vi "S_ASD Each Burst SAVE Modified_MS VI.vi"(5 "BL and Raw":T4, 7 "BCC":T1, 8 "error in":errorcluster, 9 "Under D array":T5, 10 "Burst Array":T2, 11 "Filename":path) -> (0 "error out":errorcluster, 2 "R Burst#":i32, 3 "B Table":string[][](table))   [LabVIEW 2018]
uses:
  <vilib>/Analysis/baseanly.llb/Multimode.vi
  <vilib>/Utility/file.llb/Write Delimited Spreadsheet (DBL).vi
  <vilib>/Analysis/NI_AALBase.lvlib
panel:
  out "Estimated BL":dbl[](array[numeric])
  out "B#":i32
  out "Signal# Sum":i32
  out "Burst#Sum Pre":i32
  out "B STD (pA)":dbl
  out "B BL (pA)":dbl
  out "R STD (pA)":dbl
  out "R BL (pA)":dbl
  out "BR TL Point":i32
  out "F ex Info":T3
  out "Burst time length":dbl[](array[numeric])
  in  "Flit Rank":i32=15
  out "LL BR number (n)":i32
  out "BR I-t profie":cluster{dbl[], dbl[]}[](graph)
  out "BR time length (ms)":dbl
  out "BR End time (s)":dbl
  out "BR Start time (s)":dbl
  out "BR number (n)":dbl
  out "REnd time":dbl[](array[numeric])
  out "RStart time":dbl[](array[numeric])
  out "Region Raw data":dbl[](array[numeric])
  out "BR Histogram Graph":T6(graph) caption="ヒストグラムグラフ"
  out "サイズ":i32
  out "BR END IDX":i32
  out "BR Start IDX":i32
  out "A New folder":string
  out "LL BR time length (ms)":dbl
  out "Rigon#":i32
  out "BSX Pass":path
  out "B Region":dbl[](array[numeric])
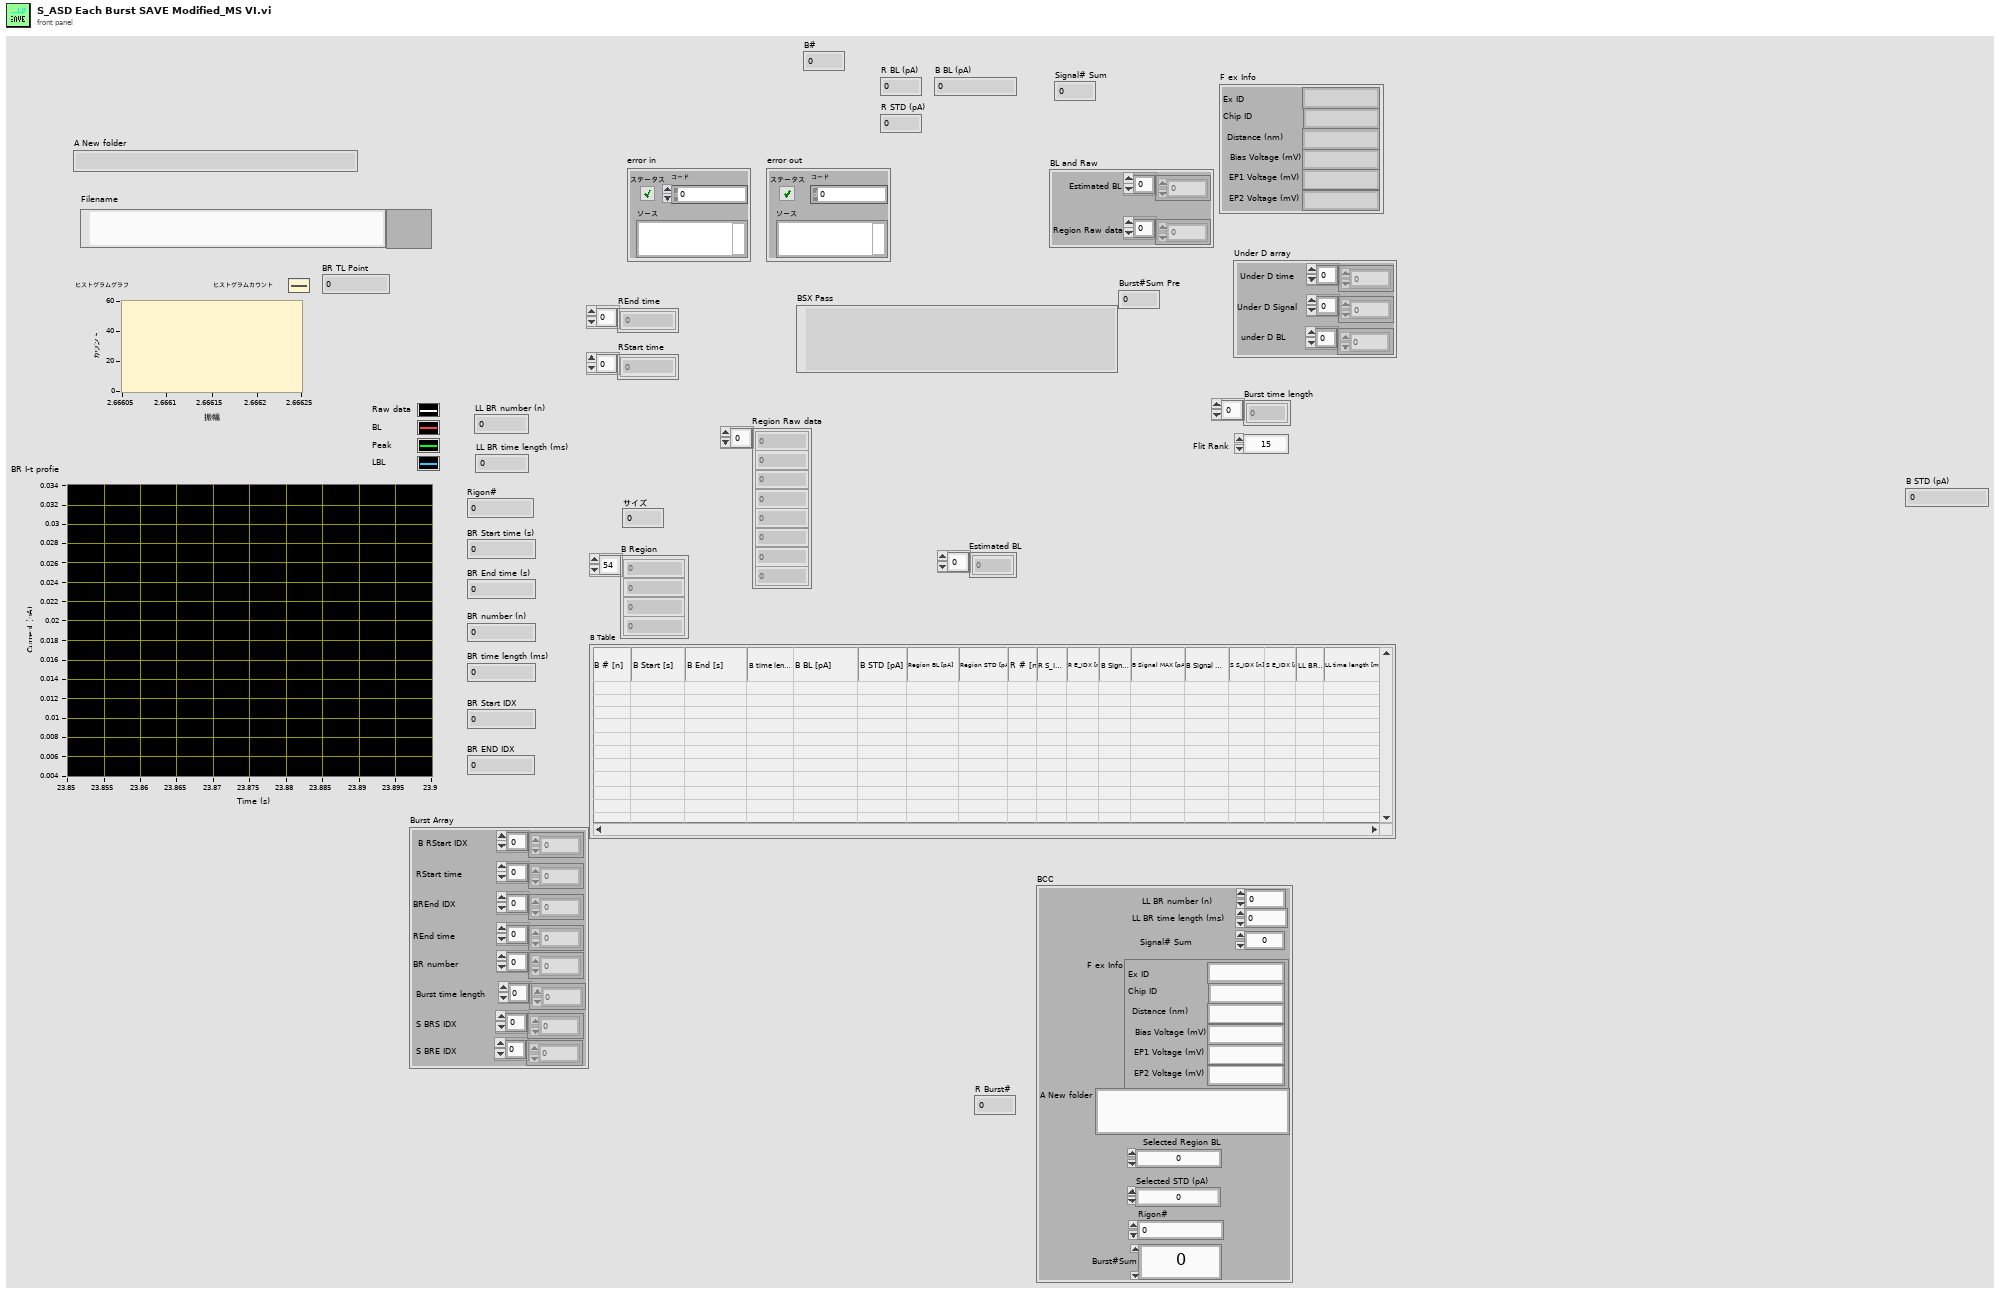
[diagram p1: front panel]
types:
  T1 = cluster{"LL BR number (n)":i32, "LL BR time length (ms)":dbl, "Signal# Sum":i32, "F ex Info":cluster{"Ex ID":string, "Chip ID":string, "Distance (nm)":string, "Bias Voltage (mV)":string, "EP1 Voltage (mV)":string, "EP2 Voltage (mV)":string}, "A New folder":string, "Selected STD (pA)":dbl, "Selected Region BL":dbl, "Rigon#":i32, "Burst#Sum":i32}
  T2 = cluster{"B RStart IDX":i32[], "RStart time":dbl[], "BREnd IDX":i32[], "REnd time":dbl[], "BR number":dbl[], "Burst time length":dbl[], "S BRS IDX":i32[], "S BRE IDX":i32[]}
  T3 = cluster{"Ex ID":string, "Chip ID":string, "Distance (nm)":string, "Bias Voltage (mV)":string, "EP1 Voltage (mV)":string, "EP2 Voltage (mV)":string}
  T4 = cluster{"Estimated BL":dbl[], "Region Raw data":dbl[]}
  T5 = cluster{"Under D time":dbl[], "Under D Signal":dbl[], "under D BL":dbl[]}
  T6 = cluster{"X Values":dbl[], "Histogram: h(x)":i32[]}
  T7 = cluster{"B Under D time":dbl[], "B Under D Signal ":dbl[], "B Under D IDX":i32[], "B Under D BL":dbl[]}
  T8 = cluster{"Size":string, "SH1":string, "SH2":string}
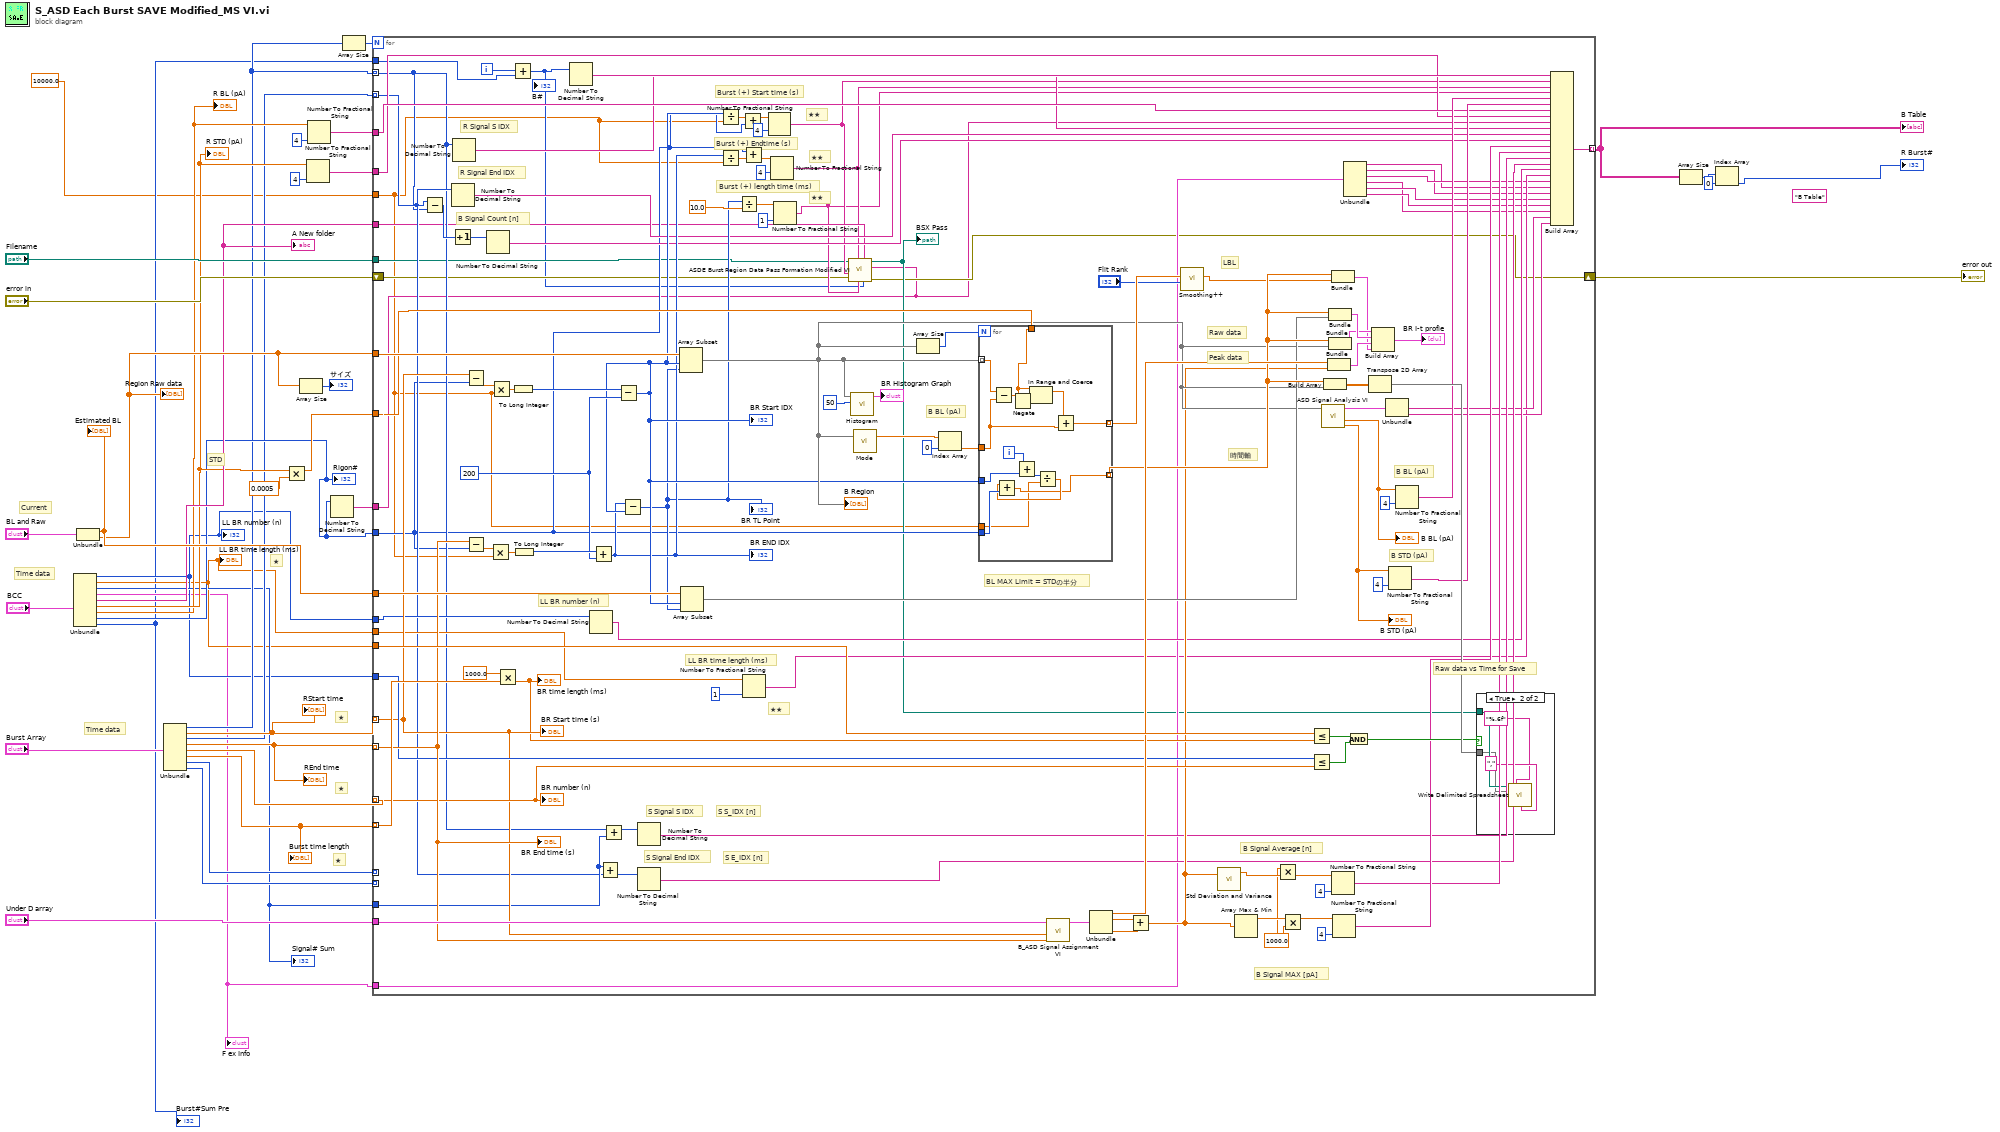
[diagram p0: block diagram]
diagram:
  (unwired) "B Table" ("Group name")
  # "★"
  # "★"
  # "★"
  # "★"
  # "Time data"
  # "Time data"
  # "Current"
  # "STD"
  n1 = Unbundle("BCC") -> ("LL BR number (n)"=w9:i32, "LL BR time length (ms)"=w8:dbl, "Signal# Sum"=w10:i32, "F ex Info"=w7:T3, "A New folder"=w23:string, "Selected STD (pA)"=w20:dbl, "Selected Region BL"=w19:dbl, "Rigon#"=w18:i32, "Burst#Sum"=w6:i32)
  "Rigon#" <- w18
  "LL BR time length (ms)" <- w8
  "A New folder" <- w23
  "LL BR number (n)" <- w9
  "F ex Info" <- w7
  "R BL (pA)" <- w19
  "R STD (pA)" <- w20
  "Burst#Sum Pre" <- w6
  "Signal# Sum" <- w10
  n2 = Unbundle("BL and Raw") -> ("Estimated BL"=w27:dbl[], "Region Raw data"=w26:dbl[])
  "Region Raw data" <- w26
  "Estimated BL" <- w27
  n3 = Unbundle("Burst Array") -> ("B RStart IDX"=w16:i32[], "RStart time"=w33:dbl[], "BREnd IDX"=w17:i32[], "REnd time"=w35:dbl[], "BR number"=w32:dbl[], "Burst time length"=w34:dbl[], "S BRS IDX"=w12:i32[], "S BRE IDX"=w11:i32[])
  "RStart time" <- w33
  "REnd time" <- w35
  "Burst time length" <- w34
  n4 = Multiply(x=w20, y=0.0005) -> (x*y=w30:dbl)
  n5 = Array Size(array=w26) -> (size(s)=→"サイズ":i32)
  n6 = Number To Fractional String(number=w20, precision (6)=i16 4 ("精度（6）")) -> (F-format string=w21:string)  [unwired: 2 in]
  n7 = Number To Fractional String(number=w19, precision (6)=i16 4 ("精度（6）")) -> (F-format string=w22:string)  [unwired: 2 in]
  n8 = Number To Decimal String(number=w18) -> (decimal integer string=w38:string)  [unwired: 1 in]
  n9 = Array Size(array=w16) -> (size(s)=w40:i32)
  n10 = for {
    N: w40 -> [_]
    tunnel: "Filename" -> [w43]
    tunnel: w26 -> [w158]
    tunnel: w38 -> [w47]
    tunnel: w18 -> [w54]
    tunnel: w8 -> [w155]
    shift-right: [w50] -> w2
    shift-left: "error in" -> [w44]
    tunnel: w23 -> [w49]
    tunnel: w33 -> [w113] mode=indexing
    tunnel: w35 -> [w131] mode=indexing
    tunnel: w34 -> [w151] mode=indexing
    tunnel: w32 -> [w129] mode=indexing
    tunnel: w27 -> [w143]
    tunnel: "Under D array" -> [w137]
    tunnel: w9 -> [w130]
    tunnel: w30 -> [w122]
    tunnel: w22 -> [w95]
    tunnel: w21 -> [w94]
    tunnel: w17 -> [w58] mode=indexing
    tunnel: w16 -> [w57] mode=indexing
    tunnel: w12 -> [_] mode=indexing
    tunnel: w11 -> [_] mode=indexing
    tunnel: w6 -> [w78]
    tunnel: w10 -> [w75]
    tunnel: w9 -> [w72]
    tunnel: w8 -> [w70]
    tunnel: w7 -> [w69]
    tunnel: [w60] -> w3 mode=indexing
    tunnel: 10000.0 ("y") -> [w41]
    i -> [w79]
    w82 = 1000.0 ("y")
    w139 = 200 ("S datapoint")
    # "★★"
    # "★★"
    # "★★"
    # "★★"
    # "LL BR time length (ms)"
    # "LL BR number (n)"
    # "S E_IDX [n]"
    # "S S_IDX [n]"
    # "S Signal End IDX"
    # "S Signal S IDX"
    # "B Signal MAX [pA]"
    # "B Signal Average [n]"
    # "B Signal Count [n]"
    # "R Signal End IDX"
    # "R Signal S IDX"
    # "B STD (pA)"
    # "B BL (pA)"
    # "B BL (pA)"
    # "Burst (+) length time (ms)"
    # "Burst (+) Endtime (s)"
    # "Burst (+) Start time (s)"
    # "BL MAX Limit = STDの半分"
    # "Peak data"
    # "Raw data vs Time for Save"
    # "Raw data"
    # "LBL"
    # "時間軸"
    n11 = Subtract(x=w58, y=w57) -> (x-y=w91:i32)
    n12 = Number To Decimal String(number=w58) -> (decimal integer string=w92:string)  [unwired: 1 in]
    n13 = Increment(x=w91) -> (x+1=w90:i32)
    n14 = Number To Decimal String(number=w57) -> (decimal integer string=w93:string)  [unwired: 1 in]
    n15 = Subtract(x=w113, y=w54) -> (x-y=w147:dbl)
    n16 = Subtract(x=w131, y=w54) -> (x-y=w146:dbl)
    n17 = Number To Decimal String(number=w90) -> (decimal integer string=w89:string)  [unwired: 1 in]
    n18 = Multiply(x=w146, y=w41) -> (x*y=w149:dbl)
    n19 = Multiply(x=w147, y=w41) -> (x*y=w150:dbl)
    n20 = Multiply(x=1000.0, y=w151) -> (x*y=w105:dbl)
    "BR time length (ms)" <- w105
    n21 = Add(x=w79, y=w78) -> (x+y=w42:i32)
    "B#" <- w42
    n22 = To Long Integer(number=w150) -> (32bit integer=w145:i32)
    n23 = To Long Integer(number=w149) -> (32bit integer=w144:i32)
    n24 = Number To Decimal String(number=w42) -> (decimal integer string=w114:string)  [unwired: 1 in]
    n25 = Number To Decimal String(number=w72) -> (decimal integer string=w71:string)  [unwired: 1 in]
    n26 = Add(x=w144, y=w139) -> (x+y=w109:i32)
    "BR END IDX" <- w109
    n27 = Add(x=w75, y=w58) -> (x+y=w76:i32)
    n28 = Add(x=w57, y=w75) -> (x+y=w77:i32)
    n29 = Subtract(x=w145, y=w139) -> (x-y=w112:i32)
    "BR Start IDX" <- w112
    n30 = Subtract(x=w109, y=w112) -> (x-y=w106:i32)
    "BR TL Point" <- w106
    n31 = Number To Decimal String(number=w76) -> (decimal integer string=w73:string)  [unwired: 1 in]
    n32 = Number To Decimal String(number=w77) -> (decimal integer string=w74:string)  [unwired: 1 in]
    n33 = Array Subset(array=w158, index=w112, length=w106) -> (w118:dbl[])
    "B Region" <- w118
    n34 = Array Subset(array=w143, index=w112, length=w106) -> (w123:dbl[])
    n35 = Divide(x=w112, y=w41) -> (x/y=w111:dbl)
    n36 = Divide(x=w109, y=w41) -> (x/y=w110:dbl)
    n37 = Divide(x=w106, y=10.0) -> (x/y=w107:dbl)
    n38 = Add(x=w111, y=w54) -> (x+y=w56:dbl)
    n39 = Add(x=w54, y=w110) -> (x+y=w55:dbl)
    n40 = Number To Fractional String(number=w70, precision (6)=i16 1 ("精度（6）")) -> (F-format string=w66:string)  [unwired: 2 in]
    n41 = Number To Fractional String(number=w56, precision (6)=i16 4 ("精度（6）")) -> (F-format string=w46:string)  [unwired: 2 in]
    n42 = Number To Fractional String(number=w55, precision (6)=i16 4 ("精度（6）")) -> (F-format string=w48:string)  [unwired: 2 in]
    n43 = Number To Fractional String(number=w107, precision (6)=i16 1 ("精度（6）")) -> (F-format string=w45:string)  [unwired: 2 in]
    n44 = call "ASDE Burst Region Data Pass Formation Modified VI.vi"("B#"=w42, "A New folder"=w49, "Burst Time (ms)"=w45, "Burst End"=w48, "error in"=w44, "Burst Start"=w46, "N #"=w47, "Filename"=w43) -> ("error out"=w50:errorcluster, "BSX Pass"=w51:path)  [unwired: 2 in]
    "BSX Pass" <- w51
    n45 = call <vilib>:"Histogram.vi"("intervals"=50, "X"=w118) -> ("Histogram Graph"=→"BR Histogram Graph":T6)  [unwired: 6 in, 3 out]
    n46 = call-poly <vilib>:"Mode.vi"("X"=w118) -> ("Modes"=w117:dbl[])  [unwired: 1 in, 1 out]
    n47 = Array Size(array=w118) -> (size(s)=w148:i32)
    n48 = Index Array(array=w117, index=0 ("指標")) -> (element=w116:dbl)
    n49 = for {
      N: w148 -> [_]
      tunnel: [w171] -> w125 mode=indexing
      tunnel: w54 -> [w174]
      tunnel: w112 -> [w173]
      tunnel: w118 -> [w170] mode=indexing
      tunnel: w116 -> [w165]
      tunnel: w122 -> [w168]
      tunnel: [w164] -> w121 mode=indexing
      tunnel: w41 -> [w163]
      i -> [w176]
      n50 = Subtract(x=w170, y=w165) -> (x-y=w169:dbl)
      n51 = Negate(x=w168) -> (-x=w167:dbl)
      n52 = Add(x=w176, y=w173) -> (x+y=w175:i32)
      n53 = In Range and Coerce(upper limit=w168, x=w169, lower limit=w167) -> (coerced(x)=w166:dbl)  [unwired: 1 out]
      n54 = Divide(x=w175, y=w163) -> (x/y=w172:dbl)
      n55 = Add(x=w172, y=w174) -> (x+y=w171:dbl)
      n56 = Add(x=w166, y=w165) -> (x+y=w164:dbl)
    }
    n57 = call "B_ASD Signal Assignment VI.vi"("BR End time (s)"=w131, "BR Start time (s)"=w113, "Under D array"=w137) -> ("Under D B Array"=w136:T7)  [unwired: 8 in]
    n58 = Unbundle(w136) -> ("B Under D time"=w135:dbl[], "B Under D Signal"=w134:dbl[], "B Under D BL"=w133:dbl[])  [unwired: 1 out]
    n59 = Add(x=w134, y=w133) -> (x+y=w88:dbl[])
    n60 = call "Smoothing++.vi"("+/- Point"="Flit Rank", "Y in"=w121) -> ("Y out"=w119:dbl[])  [unwired: 9 in]
    n61 = call <vilib>:"Std Deviation and Variance.vi"("X"=w88) -> ("mean"=w84:dbl)  [unwired: 1 in, 2 out]
    n62 = Array Max & Min(array=w88) -> (max value=w87:dbl)  [unwired: 3 out]
    n63 = Multiply(x=w82, y=w84) -> (x*y=w83:dbl)
    n64 = Multiply(x=w87, y=w82) -> (x*y=w85:dbl)
    n65 = Less Or Equal?(x=w155, y=w105) -> (x <= y?=w127:bool)
    n66 = Less Or Equal?(x=w130, y=w129) -> (x <= y?=w126:bool)
    n67 = call "ASD Signal Analysis VI.vi"("S txt"=w118) -> ("Omit STD (pA)"=w97:dbl, "BL (pA)"=w100:dbl, "S Analysis"=w154:T8)  [unwired: 8 in]
    "B BL (pA)" <- w100
    "B STD (pA)" <- w97
    n68 = Build Array(w125, w118) -> (w157:dbl[][])
    n69 = Bundle("B Under D time"=w135, w88) -> (w132:cluster{"B Under D time":dbl[], dbl[]})  [unwired: 1 in]
    n70 = Bundle(w125, w118) -> (w140:cluster{dbl[], dbl[]})  [unwired: 1 in]
    n71 = Bundle(w125, w123) -> (w141:cluster{dbl[], dbl[]})  [unwired: 1 in]
    n72 = Bundle(w125, "Y out"=w119) -> (w124:cluster{dbl[], "Y out":dbl[]})  [unwired: 1 in]
    n73 = Number To Fractional String(number=w83, precision (6)=i16 4 ("精度（6）")) -> (F-format string=w80:string)  [unwired: 2 in]
    n74 = Number To Fractional String(number=w85, precision (6)=i16 4 ("精度（6）")) -> (F-format string=w81:string)  [unwired: 2 in]
    n75 = Unbundle(w69) -> ("Ex ID"=w64:string, "Chip ID"=w63:string, "Distance (nm)"=w65:string, "Bias Voltage (mV)"=w52:string, "EP1 Voltage (mV)"=w61:string, "EP2 Voltage (mV)"=w62:string)
    n76 = And(x=w127, y=w126) -> (x .and. y?=w128:bool)
    n77 = Transpose 2D Array(2D array=w157) -> (transposed array=w156:dbl[][])
    n78 = Build Array(w140, w141, w132, w124) -> (→"BR I-t profie":cluster{"B Under D time":dbl[], "Y out":dbl[]}[])
    n79 = Unbundle(w154) -> ("SH1"=w67:string, "SH2"=w68:string)  [unwired: 1 out]
    n80 = Number To Fractional String(number=w97, precision (6)=i16 4 ("精度（6）")) -> (F-format string=w96:string)  [unwired: 2 in]
    n81 = Number To Fractional String(number=w100, precision (6)=i16 4 ("精度（6）")) -> (F-format string=w99:string)  [unwired: 2 in]
    n82 = case shown="True" w128 {
      tunnel: w51 -> [_ w162]
      tunnel: w156 -> [_ w161]
      frame False {
      }
      frame True {
        n83 = call-poly <vilib>:"Write Delimited Spreadsheet.vi"("file path (dialog if empty)"=w162, "format (%.3f)"="%.6f", "2D data"=w161, "delimiter (\\t)"="," ("delimiter (\\t)")) -> ()  [unwired: 10 in, 2 out]
      }
    }
    n84 = Build Array(w114, w46, w48, w45, w99, w96, w95, w94, w47, w93, w92, w89, w81, w80, w74, w73, w71, w66, w65, w64, w63, w61, w62, w52, w67, w68) -> (w60:string[])
    "BR number (n)" <- w129
    "BR Start time (s)" <- w113
    "BR End time (s)" <- w131
  }
  "error out" <- w2
  "B Table" <- w3
  n85 = Array Size(array=w3) -> (size(s)=w25:i32[])
  n86 = Index Array(array=w25, index=0 ("指標")) -> (element=→"R Burst#":i32)
